vi "Log Queued Error.vi"(10 "Message Data":variant) -> (0 "error out":errorcluster)   [LabVIEW 2026]
doc: "For the Error case of the main message loop: takes the Message Data variant sent by Queue-Error.vi, converts it to an error cluster and writes it to the error log with Log Error.vi.\nIf the data is not an error cluster, the conversion error itself is logged instead, so a malformed Error message is never lost silently.\nerror out reports only a failure to write the log.\n\n10/2026 Erich Schlieper"
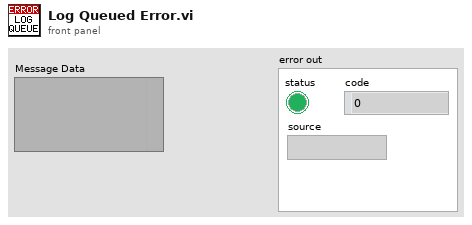
[diagram p1: front panel]
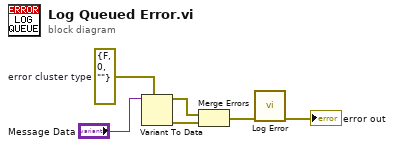
[diagram p0: block diagram]
diagram:
  w3 = errorcluster {"status"=FALSE, "code"=0, "source"=""}  # error cluster type
  n1 = Variant To Data(type=w3, Variant="Message Data") -> (data=w4:errorcluster, error out=w5:errorcluster)  [unwired: 1 in]
  n2 = Merge Errors(w4, w5) -> (w6:errorcluster)
  n3 = call "Log Error.vi"("error in"=w6) -> ("error out"=→"error out":errorcluster)  [unwired: 9 in, 1 out]
